vi "DAQ_PID.vi"() -> ()   [LabVIEW 2017]
uses:
  <userlib>/HID_ARZ/HID_ARZ.lvlib
panel:
  out "Milis":u32
  out "Conectado":bool
  in  "stop":bool
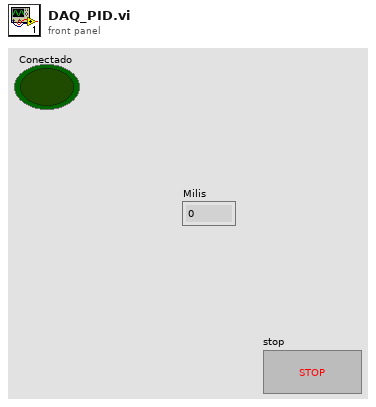
[diagram p1: front panel]
types:
  T1 = enum16{"open", "replace", "create", "open or create", "replace or create", "replace or create with confirmation"}
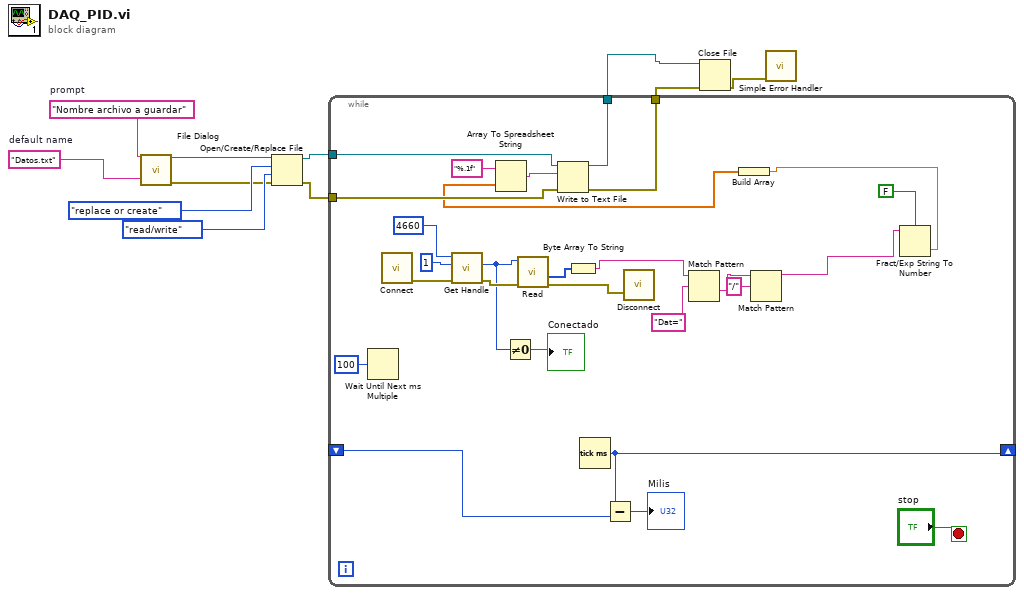
[diagram p0: block diagram]
diagram:
  w11 = "Datos.txt"  # default name
  w1 = "Nombre archivo a guardar"  # prompt
  n1 = call "File Dialog"("prompt"=w1, "pattern (all files)"=w11) -> ("selected path"=w3:path, "error out"=w2:errorcluster)  [unwired: 10 in, 2 out]
  n2 = Open/Create/Replace File(file path (use dialog)=w3, error in=w2, operation (0:open)=T1."replace or create", access (0:read/write)=enum16{"read/write", "read-only", "write-only"}."read/write") -> (refnum out=w8:refnum<file>, error out=w7:errorcluster)  [unwired: 2 in, 1 out]
  n3 = while {
    shift-right: [w29] -> _
    shift-left: _ -> [w28]
    tunnel: w8 -> [w23]
    tunnel: w7 -> [w22]
    tunnel: [w21] -> w5
    tunnel: [w20] -> w4
    stop <- "stop" stop-if-true
    n4 = Wait Until Next ms Multiple(millisecond multiple=u32 100) -> ()  [unwired: 1 out]
    n5 = call <userlib>:"Connect.vi"() -> ("error out"=w37:errorcluster)  [unwired: 9 in, 2 out]
    n6 = call <userlib>:"Get Handle.vi"("error in (no error)"=w37, "PID"=u32 1, "VID"=u32 4660) -> ("error out"=w33:errorcluster, "HANDLE"=w32:u32)  [unwired: 7 in]
    n7 = Not Equal To 0?(x=w32) -> (x != 0?=→"Conectado":bool)
    n8 = call <userlib>:"Read.vi"("error in (no error)"=w33, "HANDLE"=w32) -> ("error out"=w30:errorcluster, "BUFFER"=w31:u8[])  [unwired: 7 in, 1 out]
    n9 = Byte Array To String(unsigned byte array=w31) -> (string=w19:string)
    n10 = Tick Count (ms)() -> (millisecond timer value=w29:u32)
    n11 = Subtract(x=w29, y=w28) -> (x-y=→"Milis":u32)
    n12 = call <userlib>:"Disconnect.vi"("error in (no error)"=w30) -> ()  [unwired: 10 in, 1 out]
    n13 = Match Pattern(string=w19, regular expression="Dat=") -> (after substring=w17:string)  [unwired: 1 in, 3 out]
    n14 = Match Pattern(string=w17, regular expression="/") -> (before substring=w15:string)  [unwired: 1 in, 3 out]
    n15 = Fract/Exp String To Number(use system decimal point (T)=FALSE, string=w15) -> (number=w12:dbl)  [unwired: 2 in, 1 out]
    n16 = Build Array(w12) -> (w13:dbl[])
    n17 = Array To Spreadsheet String(array=w13, 3:"%.1f") -> (spreadsheet string=w25:string)  [unwired: 1 in]
    n18 = Write to Text File(file (use dialog)=w23, text=w25, error in=w22) -> (refnum out=w21:refnum<file>, error out=w20:errorcluster)  [unwired: 1 in, 1 out]
  }
  n19 = Close File(refnum=w5, error in=w4) -> (error out=w6:errorcluster)  [unwired: 1 out]
  n20 = call <vilib>:"Simple Error Handler.vi"("error in (no error)"=w6) -> ()  [unwired: 4 in, 5 out]
